vi "RFH-replace_name.vi"(5 "New name":string, 7 "replace":string, 11 "Filename in":string) -> (3 "Filename out":string)   [LabVIEW 2020, in "RFH-Reflection_File_Handler.lvlib"]
doc: "Replaces a text in a file name with a new name."
uses:
  RFH-Reflection_File_Handler.lvlib
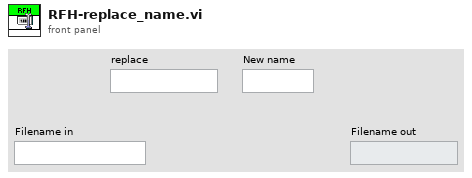
[diagram p1: front panel]
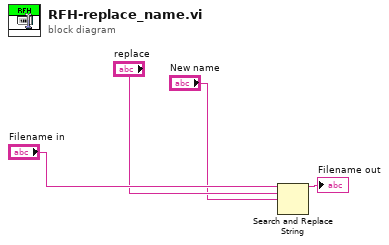
[diagram p0: block diagram]
diagram:
  n1 = Search and Replace String(input string="Filename in", search string="replace", replace string="New name") -> (result string=→"Filename out":string)  [unwired: 5 in, 3 out]
